vi "XPN Get Latest Frame.vi"(7 "height":i32, 8 "error in (no error)":errorcluster, 9 "width":i32, 10 "bufferSize":i32, 11 "lvBuffer":u16) -> (0 "error out":errorcluster, 1 "width out":i32, 2 "function return":i32, 3 "lvBuffer out":u16, 5 "height out":i32)   [LabVIEW 2025, in "xPanelWrapper.lvlib"]
doc: "XPN_API int XPN_GetLatestFrame(unsigned short* lvBuffer, int bufferSize,\n int* width, int* height);"
uses:
  xPanelWrapper.lvlib
  xPanelWrapper.dll
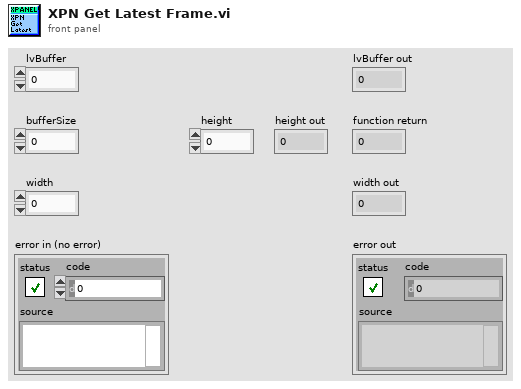
[diagram p1: front panel]
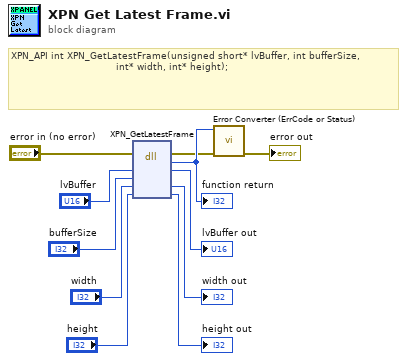
[diagram p0: block diagram]
diagram:
  # "XPN_API int XPN_GetLatestFrame(unsigned short* lvBuffer, int bufferSize,\n                                   int* width, int* height);"
  n1 = dll-call lib="E:/GitHub/xPanelWrapper/xPanelWrapperLvLib/xPanelWrapper.*" fn="XPN_GetLatestFrame"(error in="error in (no error)", "lvBuffer"="lvBuffer", "bufferSize"="bufferSize", "width"="width", "height"="height") -> (error out=w2:errorcluster, w11:i32, "lvBuffer"=→"lvBuffer out":u16, "width"=→"width out":i32, "height"=→"height out":i32)  [unwired: 3 in, 1 out]
  "function return" <- w11
  n2 = call "Error Converter (ErrCode or Status).vi"("error in (no error)"=w2, "error code"=w11) -> ("error out"=→"error out":errorcluster)  [unwired: 9 in]
